vi "attachments.get.vi"(8 "error in (no error)":errorcluster, 11 "Run in":refnum<class "Run.lvclass">) -> (0 "error out":errorcluster, 2 "attachments":string[](array[string]), 3 "Run out":refnum<class "Run.lvclass">)   [LabVIEW 2020, in "Run.lvclass"]
uses:
  Run.lvclass
  Run.lvclass/Run.ctl
  f8940fc2-285b-4416-aebd-2c1d34bf7d3c.vi
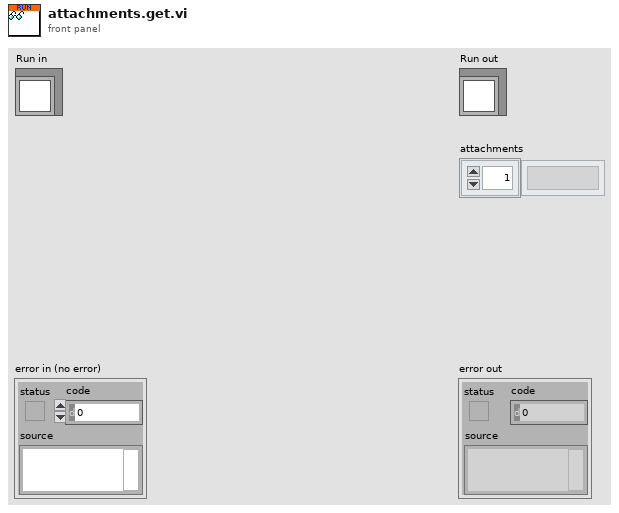
[diagram p1: front panel]
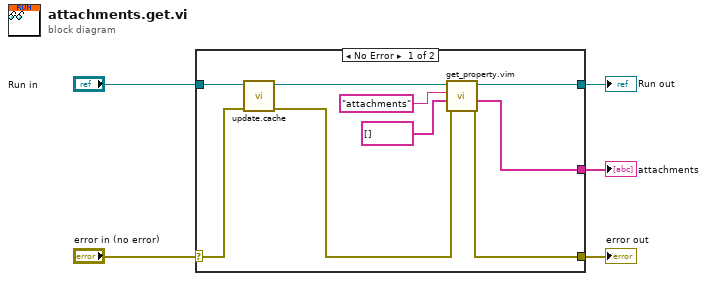
[diagram p0: block diagram]
diagram:
  n1 = case shown="No Error" "error in (no error)" {
    selector: "error in (no error)" -> [w14 w15]
    tunnel: [w6 w15] -> w4
    tunnel: [w9 w16] -> w2
    tunnel: "Run in" -> [w13 w16]
    tunnel: [w8 _] -> w1
    frame No Error {
      n2 = call "update.cache.vi"("error in"=w14, "Run in"=w13) -> ("error out"=w7:errorcluster, "Run out"=w10:refnum<class "Run.lvclass">)  [unwired: 8 in]
      n3 = call "get_property.vim"("error in"=w7, "default value and type"=string[] [] ("attachments"), "Property Name"="attachments", "Run in"=w10) -> ("error out"=w6:errorcluster, "Value"=w8:string[], "Run out"=w9:refnum<class "Run.lvclass">)  [unwired: 5 in]
    }
    frame Error {
    }
  }
  "error out" <- w4
  "Run out" <- w2
  "attachments" <- w1
